vi "Start Acq.vi"(6 "Filename":string, 8 "error in (no error)":errorcluster, 9 "Write to disk":bool, 10 "Frame Count":i32=-1, 11 "Abstract Camera Actor in":refnum<class "Abstract DAQ Triggered Actor.lvclass">) -> (0 "error out":errorcluster, 2 "File path":path, 3 "Abstract Camera Actor out":refnum<class "Abstract DAQ Triggered Actor.lvclass">)   [LabVIEW 2020, in "DAQ Timed SPIM.lvlib" / "Abstract DAQ Triggered Actor.lvlib" / "Abstract DAQ Triggered Actor.lvclass"]
uses:
  Abstract DAQ Triggered Actor.lvclass
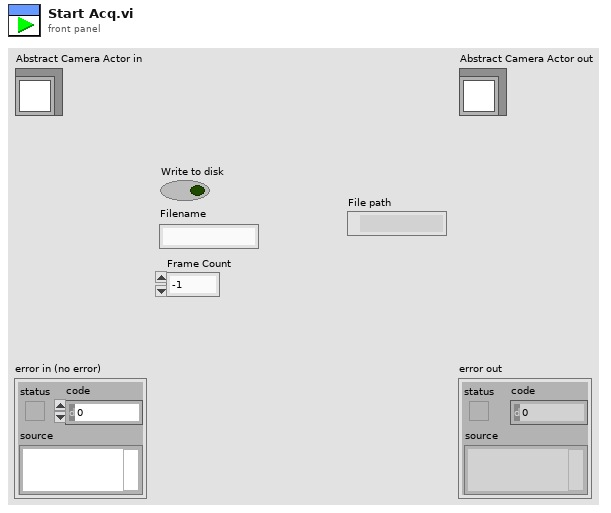
[diagram p1: front panel]
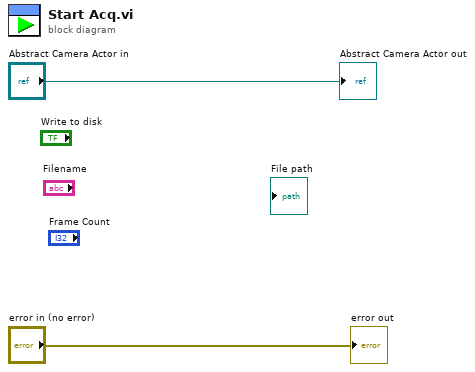
[diagram p0: block diagram]
diagram:
  "error out" <- "error in (no error)"
  "Abstract Camera Actor out" <- "Abstract Camera Actor in"
